vi "Sim_Data.vi"(11 "Number in":i32) -> (3 "data":dbl[][](array[numeric]))   [LabVIEW 2025]
uses:
  <vilib>/Analysis/NI_AALBase.lvlib
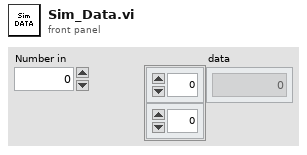
[diagram p1: front panel]
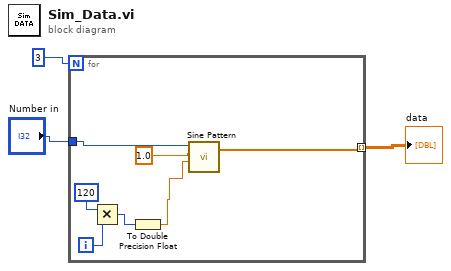
[diagram p0: block diagram]
diagram:
  n1 = for {
    N: 3 -> [_]
    tunnel: "Number in" -> [w10]
    tunnel: [w4] -> w3 mode=indexing
    i -> [w8]
    n2 = Multiply(x=120, y=w8) -> (x*y=w6:i32)
    n3 = To Double Precision Float(number=w6) -> (double precision float=w5:dbl)
    n4 = call <vilib>:"Sine Pattern.vi"("phase(degrees)"=w5, "amplitude"=1.0, "samples"=w10) -> ("Sinusoidal Pattern"=w4:dbl[])  [unwired: 1 in, 1 out]
  }
  "data" <- w3
